vi "Header.vi"() -> ()   [LabVIEW 2013]
uses:
  <vilib>/Utility/miscctls.llb/LVPointTypeDef.ctl
  Globals/Global VI.vi
  Globals/Global Recipe.vi
panel:
  out "Recipe":string="Recipe_1"
  out "System Status :":u16(ring)=5 items=["NOT READY", "E-STOPPED", "FAULTED", "PAUSING...", "PAUSED", "IDLE", "RUNNING", "UNCALIBRATED", "CALIBRATING...", "POWER OFF", "POWERING ON...", "MANUAL MODE", "CONNECTING..."]
  out "Faulted":bool
  in  "Previous Button":bool
  in  "Next Button":bool
  in  "Last Button":bool
  in  "First Button":bool
  in  "Login Button":bool
  out "Date/Time":string="Monday\n08/08/2011\n11:41:14 AM"
  out "String":string="Recipe"
  out "Operator":string="Operator"
  out "System Info":string="System Idle"
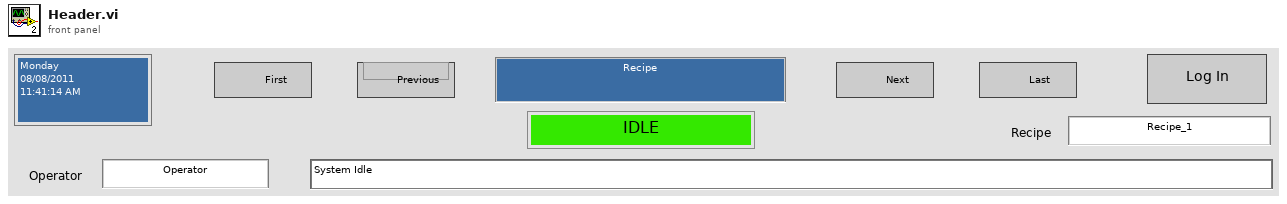
[diagram p1: front panel]
types:
  T1 = typedef "LVPointTypeDef.ctl" = cluster{"Horizontal":i16, "Vertical":i16}
  T2 = enum16{"Always On", "Always Off", "Off While Running"}
  T3 = typedef "LVAllMonitorsDisplayTypeDef.ctl" = cluster{"Bounds":cluster{"Left":i16, "Top":i16, "Right":i16, "Bottom":i16}, "Depth":i16}[]
  T4 = typedef "LVRectTypeDef.ctl" = cluster{"Left":i16, "Top":i16, "Right":i16, "Bottom":i16}
  T5 = cluster{"Bounds":cluster{"Left":i16, "Top":i16, "Right":i16, "Bottom":i16}, "Depth":i16}
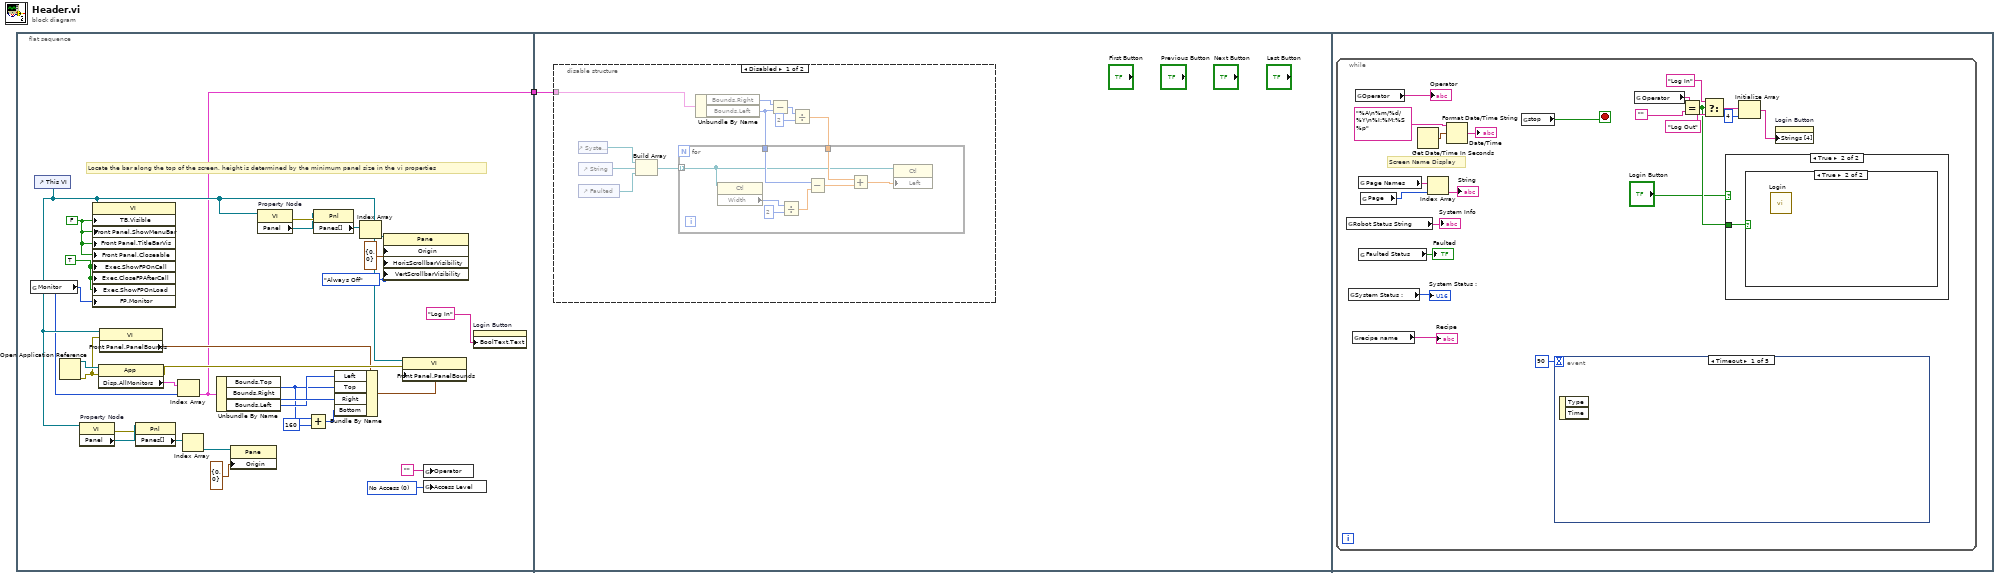
[diagram p0: block diagram]
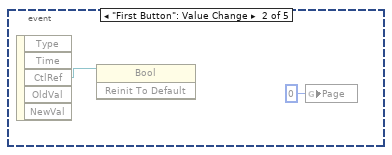
[diagram p3: hidden frame]
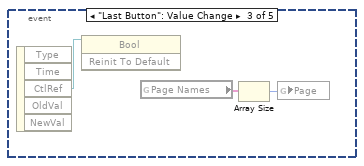
[diagram p4: hidden frame]
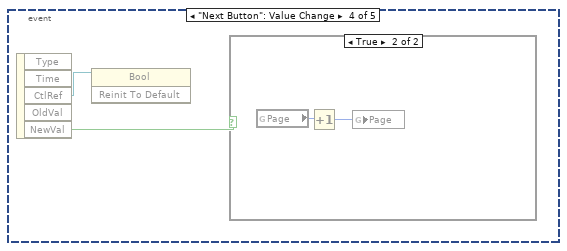
[diagram p5: hidden frame]
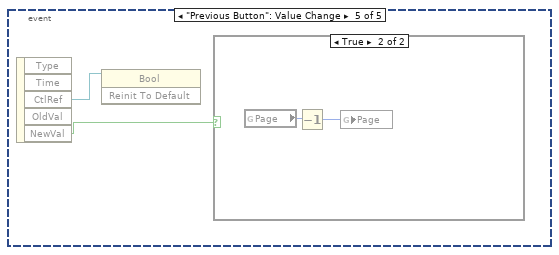
[diagram p7: hidden frame]
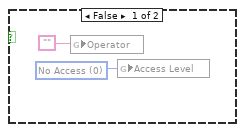
[diagram p10: hidden frame]
diagram:
  n1 = flat-sequence {
    tunnel: [w3] -> w1
    tunnel: w1 -> [w32]
    frame #0 {
      w6 = u16 0 items=["No Access", "Operator", "Engineer/Tech"] ("Access Level")
      w9 = TRUE ("Execution:Show Front Panel On Call")
      w8 = FALSE ("Tool Bar:Visible")
      w11 = T2."Always Off" ("Horizontal Scrollbar Visibility")
      # "Locate the bar along the top of the screen, height is determined by the minimum panel size in the vi properties"
      n2 = global read "Global VI.vi" "Monitor"() -> (w2:u16)
      n3 = control-ref of="This VI"() -> (w7:refnum<vi>)
      n4 = Open Application Reference() -> (0:w27:errorcluster, 3:w28:refnum<vi>)  [unwired: 4 in]
      n5 = property on="Property Node" class="VI"(reference=w7) -> (error out=w25:errorcluster, "Panel"=w26:refnum<vi>)  [unwired: 1 in, 1 out]
      n6 = property class="VI"(reference=w7, "TB.Visible"=w8, "Front Panel.ShowMenuBar"=w8, "Front Panel.TitleBarVis"=w8, "Front Panel.Closeable"=w8, "Exec.ShowFPOnCall"=w9, "Exec.CloseFPAfterCall"=w9, "Exec.ShowFPOnLoad"=w9, "FP.Monitor"=w2) -> ()  [unwired: 1 in, 2 out]
      n7 = property class="App"(reference=w28, error in=w27) -> (error out=w30:errorcluster, "Disp.AllMonitors"=w31:T3)  [unwired: 1 out]
      n8 = property class="VI"(reference=w7, error in=w27) -> ("Front Panel.PanelBounds"=w21:T4)  [unwired: 2 out]
      n9 = property class="Pnl"(reference=w26, error in=w25) -> ("Panes[]"=w24:refnum<vi>[])  [unwired: 2 out]
      n10 = Index Array(array=w31, index=w2) -> (element=w3:T5)
      n11 = Index Array "Index Array"(array=w24) -> (element=w23:refnum<vi>)  [unwired: 1 in]
      n12 = Unbundle By Name(w3) -> ("Bounds.Top"=w18:i16, "Bounds.Right"=w20:i16, "Bounds.Left"=w19:i16)
      n13 = property class="Pane"(reference=w23, "Origin"=T1 {"Horizontal"=0, "Vertical"=0}) -> ()  [unwired: 1 in, 2 out]
      n14 = property on="Property Node" class="VI"(reference=w7) -> (error out=w13:errorcluster, "Panel"=w12:refnum<vi>)  [unwired: 1 in, 1 out]
      n15 = Add(x=w18, y=i16 160) -> (x+y=w16:i16)
      n16 = property class="Pnl"(reference=w12, error in=w13) -> ("Panes[]"=w14:refnum<vi>[])  [unwired: 2 out]
      n17 = Bundle By Name(cluster=w21, "Left"=w19, "Top"=w18, "Right"=w20, "Bottom"=w16) -> (w29:T4)
      n18 = Index Array "Index Array"(array=w14) -> (element=w15:refnum<vi>)  [unwired: 1 in]
      n19 = property class="Pane"(reference=w15, "Origin"=T1 {"Horizontal"=0, "Vertical"=0}, "HorizScrollbarVisibility"=w11, "VertScrollbarVisibility"=w11) -> ()  [unwired: 1 in, 2 out]
      n20 = property on="Property Node" class="VI"(reference=w7, error in=w30, "Front Panel.PanelBounds"=w29) -> ()  [unwired: 2 out]
      n21 = global write "Global VI.vi" "Operator"("") -> ()
      n22 = global write "Global VI.vi" "Access Level"(w6) -> ()
      n23 = property on="Login Button" class="Bool"("BoolText.Text"="Log In" ("Boolean Text.Text")) -> ()  [unwired: 2 in, 2 out]
    }
    frame #1 {
      n24 = disable-structure shown="Disabled" {
        disable-tunnel: w32 -> [w39 _]
        frame Disabled {
          n25 = control-ref of="System Status :"() -> (w36:refnum<vi>)
          n26 = control-ref of="Faulted"() -> (w34:refnum<vi>)
          n27 = control-ref of="String"() -> (w35:refnum<vi>)
          n28 = Build Array(w36, w35, w34) -> (w33:refnum<vi>[])
          n29 = Unbundle By Name(w39) -> ("Bounds.Right"=w40:i16, "Bounds.Left"=w37:i16)
          n30 = Subtract(x=w40, y=w37) -> (x-y=w42:i16)
          n31 = Divide(x=w42, y=u32 2) -> (x/y=w38:dbl)
          n32 = for {
            tunnel: w38 -> [w45]
            tunnel: w37 -> [w44]
            tunnel: w33 -> [w43] mode=indexing
            n33 = property class="Ctl"(reference=w43) -> ("Width"=w49:u32)  [unwired: 1 in, 2 out]
            n34 = Divide(x=w49, y=u32 2) -> (x/y=w48:dbl)
            n35 = Subtract(x=w44, y=w48) -> (x-y=w47:dbl)
            n36 = Add(x=w45, y=w47) -> (x+y=w46:dbl)
            n37 = property class="Ctl"(reference=w43, "Left"=w46) -> ()  [unwired: 1 in, 2 out]
          }
        }
        frame Enabled {
        }
      }
    }
    frame #2 {
      n38 = while {
        stop <- w63 stop-if-true
        # "Screen Name Display"
        n39 = global read "Global VI.vi" "Robot Status String"() -> (→"System Info":string)
        n40 = global read "Global Recipe.vi" "System Status :"() -> (→"System Status :":u16)
        n41 = global read "Global Recipe.vi" "recipe name"() -> (→"Recipe":string)
        n42 = global read "Global VI.vi" "Operator"() -> (→"Operator":string)
        n43 = global read "Global VI.vi" "Page Names"() -> (w69:string[])
        n44 = global read "Global VI.vi" "Faulted Status"() -> (→"Faulted":bool)
        n45 = global read "Global VI.vi" "Page"() -> (w68:i16)
        n46 = Get Date/Time In Seconds() -> (seconds since 1Jan1904=w72:timestamp)
        n47 = Index Array(array=w69, index=w68) -> (element=→"String":string)
        n48 = Format Date/Time String(time format string (%c)="%A\n%m/%d/%Y\n%I:%M:%S %p" ("HMI Date Format String"), seconds (now)=w72) -> (date/time string=→"Date/Time":string)  [unwired: 1 in]
        n49 = global read "Global VI.vi" "stop"() -> (w63:bool)
        n50 = event shown="[0] Timeout" {
          selector: _ -> [_ _ _ _ _]
          dyn-events: _ -> [_ _ _ _ _]
          timeout: 90 -> [_ _ _ _ _]
          event Timeout {
            n51 = event-data() -> ()  [unwired: 1 in, 2 out]
          }
          event "First Button": Value Change {
            n52 = event-data() -> ("CtlRef"=w73:refnum<vi>)  [unwired: 1 in, 4 out]
            n53 = invoke class="Bool" method="Reinit To Default"(reference=w73) -> ()  [unwired: 2 in, 3 out]
            n54 = global write "Global VI.vi" "Page"(i16 0 ("Page")) -> ()
          }
          event "Last Button": Value Change {
            n55 = event-data() -> ("CtlRef"=w75:refnum<vi>)  [unwired: 1 in, 4 out]
            n56 = invoke class="Bool" method="Reinit To Default"(reference=w75) -> ()  [unwired: 2 in, 3 out]
            n57 = global read "Global VI.vi" "Page Names"() -> (w76:string[])
            n58 = Array Size(array=w76) -> (size(s)=w77:i32)
            n59 = global write "Global VI.vi" "Page"(w77) -> ()
          }
          event "Next Button": Value Change {
            n60 = event-data() -> ("CtlRef"=w78:refnum<vi>, "NewVal"=w79:bool)  [unwired: 1 in, 3 out]
            n61 = invoke class="Bool" method="Reinit To Default"(reference=w78) -> ()  [unwired: 2 in, 3 out]
            n62 = case shown="True" w79 {
              frame False {
              }
              frame True {
                n63 = global read "Global VI.vi" "Page"() -> (w81:i16)
                n64 = Increment(x=w81) -> (x+1=w80:i16)
                n65 = global write "Global VI.vi" "Page"(w80) -> ()
              }
            }
          }
          event "Previous Button": Value Change {
            n66 = event-data() -> ("CtlRef"=w82:refnum<vi>, "NewVal"=w83:bool)  [unwired: 1 in, 3 out]
            n67 = invoke class="Bool" method="Reinit To Default"(reference=w82) -> ()  [unwired: 2 in, 3 out]
            n68 = case shown="True" w83 {
              frame False {
              }
              frame True {
                n69 = global read "Global VI.vi" "Page"() -> (w85:i16)
                n70 = Decrement(x=w85) -> (x-1=w84:i16)
                n71 = global write "Global VI.vi" "Page"(w84) -> ()
              }
            }
          }
        }
        n72 = global read "Global VI.vi" "Operator"() -> (w61:string)
        n73 = Equal?(x=w61, y="") -> (x = y?=w56:bool)
        n74 = Select(t="Log In" ("Robot Status String"), s=w56, f="Log Out") -> (s? t:f=w59:string)
        n75 = case shown="True" "Login Button" {
          tunnel: w56 -> [_ w86]
          frame False {
          }
          frame True {
            n76 = case shown="True" w86 {
              frame False {
                w87 = u16 0 items=["No Access", "Operator", "Engineer/Tech"] ("Access Level")
                n77 = global write "Global VI.vi" "Operator"("") -> ()
                n78 = global write "Global VI.vi" "Access Level"(w87) -> ()
              }
              frame True {
                n79 = call "Login.vi"() -> ()  [unwired: 12 in]
              }
            }
          }
        }
        n80 = Initialize Array(w59, 4 ("dimension size")) -> (w55:string[])
        n81 = property on="Login Button" class="Bool"("Strings [4]"=w55) -> ()  [unwired: 2 in, 2 out]
      }
    }
  }
